vi "Initialize Locations.vi"(8 "error in":errorcluster, 11 "Save Location":path) -> (0 "error out":errorcluster, 3 "Archivist out":refnum<class "Archivist.lvclass">)   [LabVIEW 2019, in "Archivist.lvclass"]
uses:
  Archivist.lvclass
  Archivist.lvclass/Archivist.ctl
panel:
  out "Writing":map{string, path}(c390)
  out "Reading":map{string, path}(c390)
  in  "Archivist in":refnum<class "Archivist.lvclass">
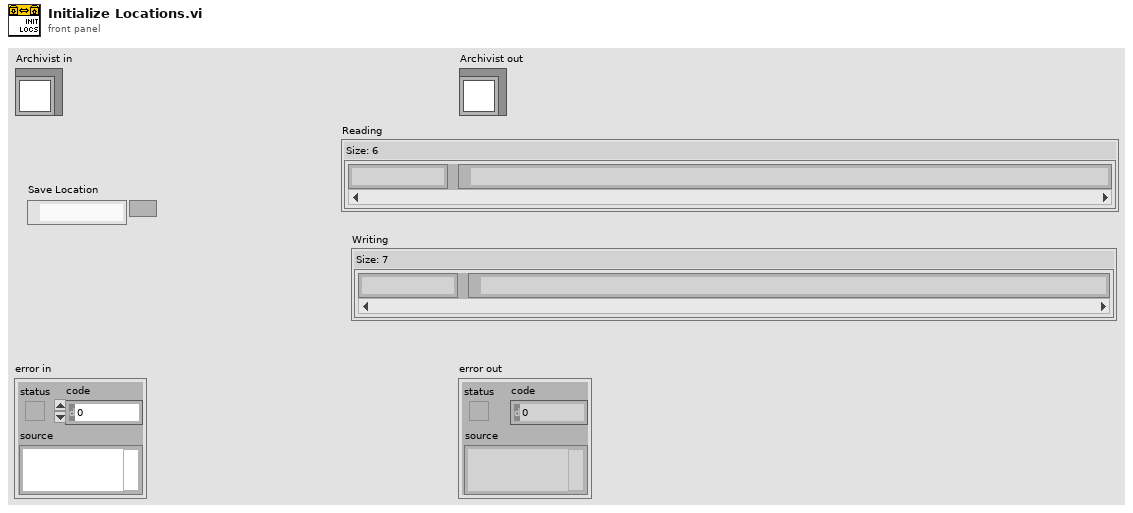
[diagram p1: front panel]
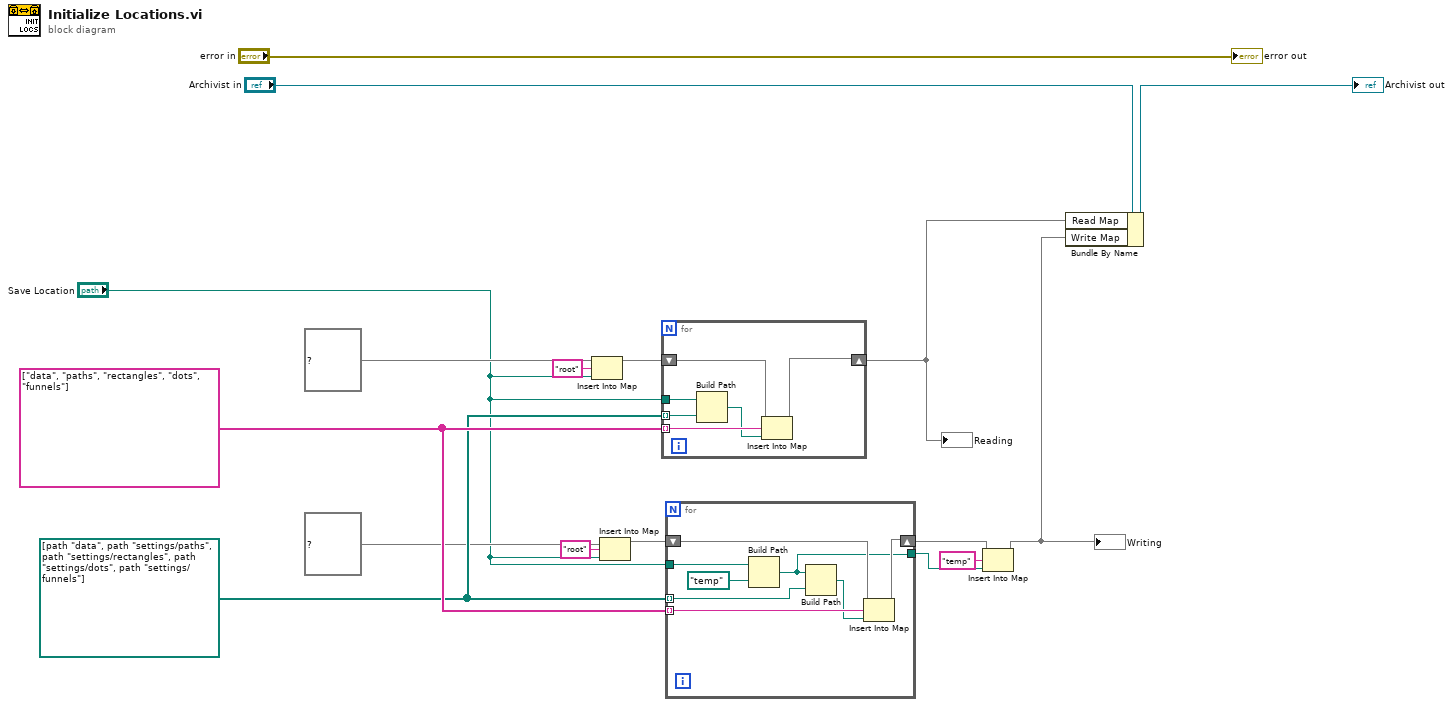
[diagram p0: block diagram]
diagram:
  w15 = path[] [path "data", path "settings/paths", path "settings/rectangles", path "settings/dots", path "settings/funnels"]
  w16 = string[] ["data", "paths", "rectangles", "dots", "funnels"]
  n1 = Insert Into Map(map in=map{string, path} {} ("map out"), key="root", value="Save Location") -> (map out=w9:map{string, path})  [unwired: 2 out]
  n2 = Insert Into Map(map in=map{string, path} {}, key="root", value="Save Location") -> (map out=w14:map{string, path})  [unwired: 2 out]
  n3 = for {
    shift-right: [w22] -> w2
    shift-left: w9 -> [w23]
    tunnel: w15 -> [w19] mode=indexing
    tunnel: w16 -> [w21] mode=indexing
    tunnel: "Save Location" -> [w20]
    n4 = Build Path(base path=w20, name or relative path=w19) -> (appended path=w18:path)
    n5 = Insert Into Map(map in=w23, key=w21, value=w18) -> (map out=w22:map{string, path})  [unwired: 2 out]
  }
  "Reading" <- w2
  n6 = for {
    shift-right: [w30] -> w5
    shift-left: w14 -> [w31]
    tunnel: w15 -> [w25] mode=indexing
    tunnel: w16 -> [w29] mode=indexing
    tunnel: "Save Location" -> [w28]
    tunnel: [w24] -> w7
    n7 = Build Path(base path=w28, name or relative path=path "temp" ("Save Location")) -> (appended path=w24:path)
    n8 = Build Path(base path=w24, name or relative path=w25) -> (appended path=w26:path)
    n9 = Insert Into Map(map in=w31, key=w29, value=w26) -> (map out=w30:map{string, path})  [unwired: 2 out]
  }
  n10 = Insert Into Map(map in=w5, key="temp", value=w7) -> (map out=w1:map{string, path})  [unwired: 2 out]
  "Writing" <- w1
  n11 = Bundle By Name(cluster="Archivist in", "Read Map"=w2, "Write Map"=w1) -> (→"Archivist out":refnum<class "Archivist.lvclass">)
  "error out" <- "error in"
